vi "Append Text Table to Report.vi"(0 "report in":refnum<class "ooWriter.lvclass">, 1 "column width (1)":dbl=1.0 format="%.2f", 2 "measurement system":u16(ring)=2 caption="measurement system for column width (Default)" items=["US", "Metric", "Default"], 3 "MS Office parameters":T2, 5 "column headers":string[](array[string]), 7 "row headers":string[](array[string]), 9 "text data":string[][](array[string]), 11 "error in (no error)":errorcluster, 13 "separate page?":bool, 14 "show grid lines":bool=TRUE) -> (4 "report out":refnum<class "ooWriter.lvclass">, 8 "range (wd) - start (xl)":T1, 10 "end (xl)":cluster{"row (xl) ":i32, "col (xl) ":i32}, 15 "error out":errorcluster)   [LabVIEW 2009, in "ooWriter.lvclass"]
doc: "Appends a 2D array to a report as a table with the given column width. You can use this polymorphic VI to append an array of strings or numbers. The data type you wire to the <B>text data</B> input determines the polymorphic instance to use."
uses:
  ooWriter.lvclass
  C:/Projets/LAVAG/OpenOfficeRGT/AODL/DLLs/AODL.dll
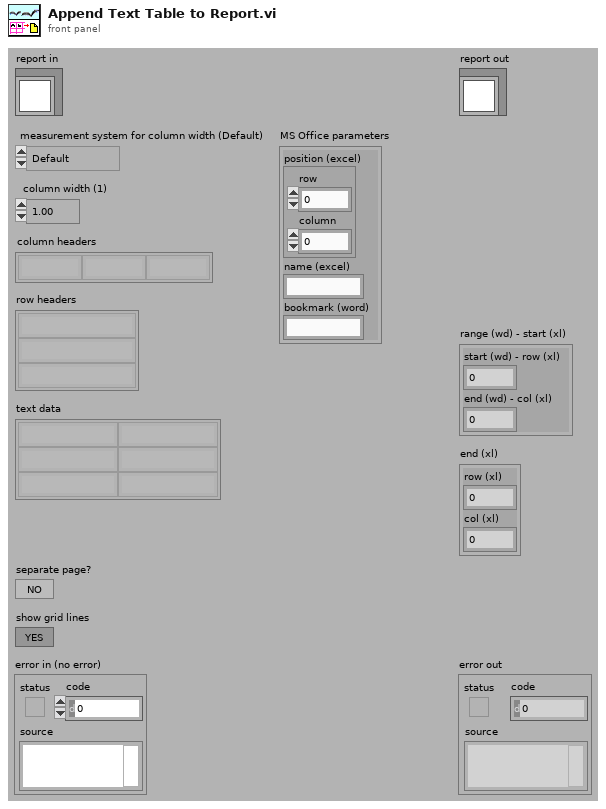
[diagram p1: front panel]
types:
  T1 = cluster{"start (wd) - row (xl) ":i32, "end (wd) - col (xl) ":i32}
  T2 = cluster{"position (excel)":cluster{"row":i32, "column":i32}, "name (excel)":string, "bookmark (word)":string}
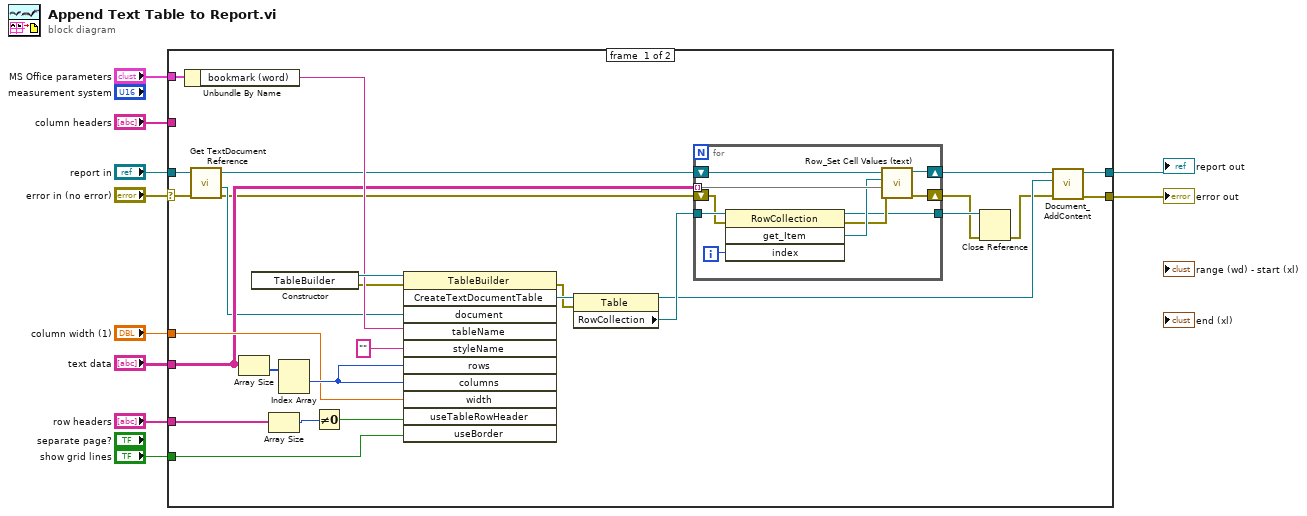
[diagram p0: block diagram]
diagram:
  n1 = case shown="No Error" "error in (no error)" {
    selector: "error in (no error)" -> [w18 w49]
    tunnel: [w25 w49] -> w9
    tunnel: "report in" -> [w16 w50]
    tunnel: [w26 w50] -> w7
    tunnel: "show grid lines" -> [w35 _]
    tunnel: "text data" -> [w23 _]
    tunnel: "column width (1)" -> [w32 _]
    tunnel: "MS Office parameters" -> [w31 _]
    tunnel: "column headers" -> [_ _]
    tunnel: "row headers" -> [w28 _]
    frame #0 {
      n2 = Unbundle By Name(w31) -> ("bookmark (word)"=w30:string)
      n3 = call-dynamic "Get TextDocument Reference.vi"("error in (no error)"=w18, "ooWriter in"=w16) -> ("error out"=w17:errorcluster, "Document"=w20:refnum<k24>, "ooWriter out"=w19:refnum<class "ooWriter.lvclass">)  [unwired: 7 in]
      n4 = Array Size(array=w23) -> (size(s)=w34:i32[])
      n5 = constructor class="TableBuilder"() -> (reference out=w38:refnum<k24>, error out=w15:errorcluster)  [unwired: 3 in, 1 out]
      n6 = Array Size(array=w28) -> (size(s)=w37:i32)
      n7 = Index Array(array=w34) -> (element #1=w33:i32)  [unwired: 2 in, 1 out]
      n8 = Not Equal To 0?(x=w37) -> (x != 0?=w36:bool)
      n9 = invoke class="TableBuilder" method="CreateTextDocumentTable"(reference=w38, error in=w15, "document"=w20, "tableName"=w30, "styleName"="", "rows"=w33, "columns"=w33, "width"=w32, "useTableRowHeader"=w36, "useBorder"=w35) -> (error out=w14:errorcluster, "CreateTextDocumentTable"=w27:refnum<k24>)  [unwired: 1 in, 9 out]
      n10 = property class="Table"(reference=w27, error in=w14) -> (reference out=w21:refnum<k24>, "RowCollection"=w22:refnum<k24>)  [unwired: 1 out]
      n11 = for {
        shift-right: [w47] -> w24
        shift-left: w19 -> [w48]
        tunnel: w23 -> [w46] mode=indexing
        tunnel: w22 -> [w44]
        shift-right: [w41] -> w12
        shift-left: w17 -> [w40]
        tunnel: [w39] -> w13
        i -> [w45]
        n12 = invoke class="RowCollection" method="get_Item"(reference=w44, error in=w40, "index"=w45) -> (reference out=w39:refnum<k24>, error out=w42:errorcluster, "get_Item"=w43:refnum<k24>)  [unwired: 1 in, 1 out]
        n13 = call-dynamic "Row_Set Cell Values (text).vi"("error in (no error)"=w42, "text data (row)"=w46, "Row"=w43, "ooWriter in"=w48) -> ("error out"=w41:errorcluster, "ooWriter out"=w47:refnum<class "ooWriter.lvclass">)  [unwired: 6 in]
      }
      n14 = Close Reference(reference=w13, error in (no error)=w12) -> (error out=w11:errorcluster)
      n15 = call-dynamic "Document_AddContent.vi"("error in (no error)"=w11, "Content"=w21, "ooWriter in"=w24) -> ("error out"=w25:errorcluster, "ooWriter out"=w26:refnum<class "ooWriter.lvclass">)  [unwired: 7 in]
    }
    frame #1 {
    }
  }
  "error out" <- w9
  "report out" <- w7
